vi "LoadMouseLUT.vi"(11 "Metadata":T3[](array[typedef])) -> (0 "error out":errorcluster)   [LabVIEW 2026, in "dependencies.lvlib"]
uses:
  dependencies.lvlib
  MouseLUTSelector.ctl
  KeyboardAndMouseDataAcquisition.ctl
  KeyType.ctl
panel:
  out "Axis Info Debug":T1(array[cluster])
  out "Button Info Debug":T2(array[cluster])
  # "wqeeeeeeeeeeeeeeeeeeeeeeeeeeeeeeeeeeeeeeeeeeeeeeeeeeeeeeeeeeeeeeeeeeeeeeeeeeeeee"
  # "sssssssssssssddddddddddddddddddddddddddddddddddddddddddd"
  # "fsdsdsdsdsdsdsdsdsdsdaaaaaaaaaaaaaaaaaaaaaaaaaaaaaaaaa"
  # "qweeeeeeeeewqqqqqqqqqqqqqqqqqqqqqqqqqqqqqqqqqqqqqqqqqq"
  # "sdffffffffffffffffffAAAAAA"
  # "sdsdsdsdsdsdsdsdsdsdaaaaaaaaaaaaaaaaaaaaaaaaaaaaaaaaaaaaaaaaaaaaaaaaaaaaaaaaaaa"
  # "rewwwwwwwwwwwwwwwwwwwwrewwerrrrrrrrrewwwwwwwwwwwwww"
  # "rew"
  # "rrrrrrrrreeeeeeeewwwwwwwwww"
  # "rrrrrrrreeeeeeeeeeewwwwwwwwwwwwwww"
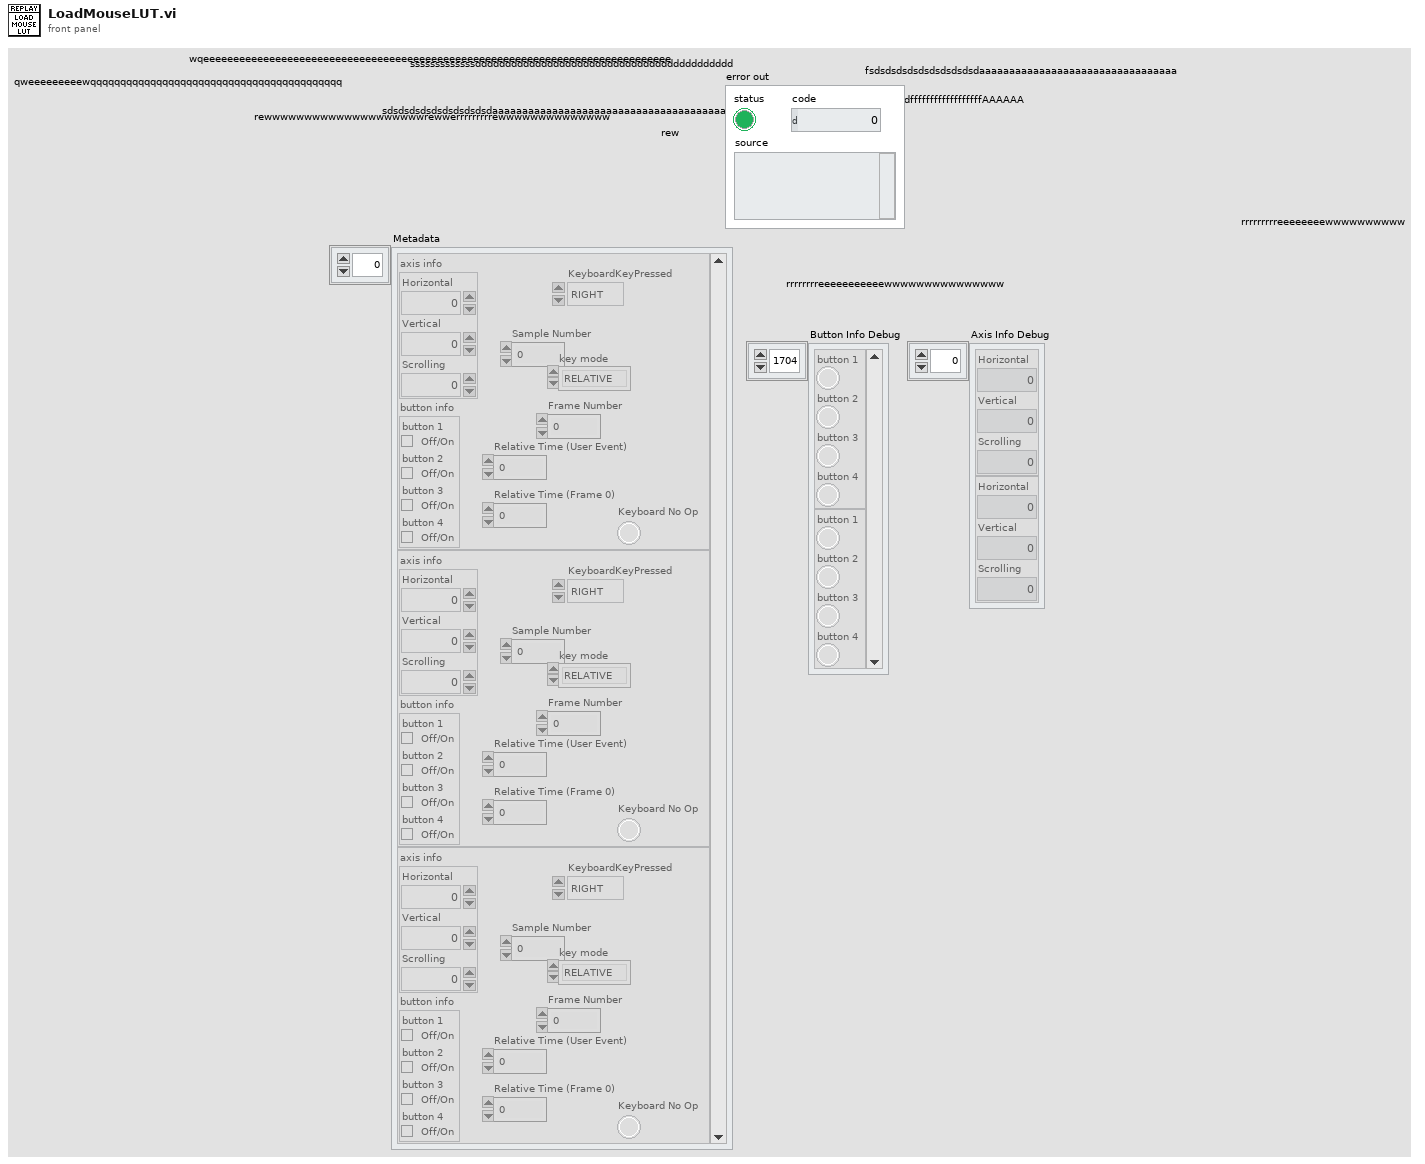
[diagram p1: front panel]
types:
  T1 = cluster{"Horizontal":i32, "Vertical":i32, "Scrolling":i32}[]
  T2 = cluster{"button 1":bool, "button 2":bool, "button 3":bool, "button 4":bool}[]
  T3 = typedef "dependencies.lvlib/KeyboardAndMouseDataAcquisition.ctl" = cluster{"axis info":cluster{"Horizontal":i32, "Vertical":i32, "Scrolling":i32}, "button info":cluster{"button 1":bool, "button 2":bool, "button 3":bool, "button 4":bool}, "Relative Time (User Event)":dbl, "Sample Number":u32, "Relative Time (Frame 0)":dbl, "key mode":enum16{"RELATIVE", "ABSOLUTE"}, "Frame Number":u32, "KeyboardKeyPressed":T4, "Keyboard No Op":bool}
  T4 = typedef "dependencies.lvlib/KeyType.ctl" = enum16{"0", "1", "2", "3", "4", "5", "6", "7", "8", "9", "A", "B", "C", "D", "E", "F", "G", "H", "I", "J", "K", "L", "M", "N", "O", "P", "Q", "R", "S", "T", "U", "V", "W", "X", "Y", "Z", "F1", "F2", "F3", "F4", "F5", "F6", "F7", "F8", "F9", "F10", "F11", "F12", "F13", "F14", "F15", "ADD", "BACK", "BACKSLASH", "CAPITAL", "COMMA", "DECIMAL", "DELETE", "DIVIDE", "DOWN", "END", "EQUALS", "ESCAPE", "GRAVE (`)", "HOME", "INSERT", "LBRACKET", "LCONTROL", "LEFT", "L ALT", "LSHIFT", "LWIN", "MINUS", "MULTIPLY", "NEXT", "NUMLOCK", "NUMPAD_0", "NUMPAD_1", "NUMPAD_2", "NUMPAD_3", "NUMPAD_4", "NUMPAD_5", "NUMPAD_6", "NUMPAD_7", "NUMPAD_8", "NUMPAD_9", "PAUSE", "PERIOD", "PRIOR (PG UP)", "RBRACKET", "RCONTROL", "RETURN", "RIGHT", "R ALT", "RSHIFT", "RWIN", "SCROLL", "SEMICOLON", "SLASH", "SPACE", "SUBTRACT", "TAB", "UP", "ENTER (num pad)", "' (quote)"}
  T5 = typedef "dependencies.lvlib/MouseLUTSelector.ctl" = enum16{"Initialize", "Get Button and Axis Info", "Assign Button and Axis Info to Sample Number"}
  T6 = cluster{"Horizontal":i32, "Vertical":i32, "Scrolling":i32}
  T7 = cluster{"button 1":bool, "button 2":bool, "button 3":bool, "button 4":bool}
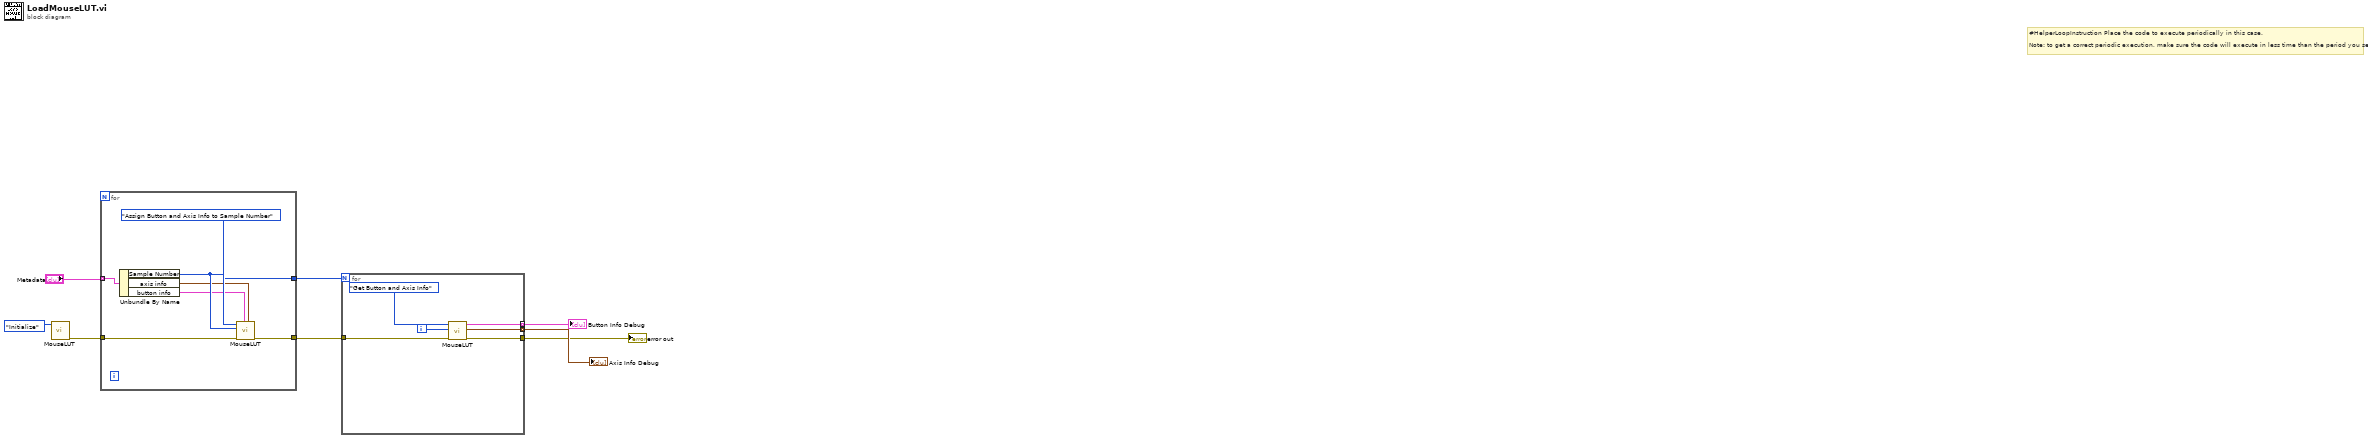
[diagram p0: block diagram]
diagram:
  # "#HelperLoopInstruction Place the code to execute periodically in this case.\n\nNote: to get a correct periodic execution, make sure the code will execute in less time than the period you set."
  n1 = call "MouseLUT.vi"("LUT Selector"=MouseLUTSelector."Initialize") -> ("error out"=w6:errorcluster)  [unwired: 8 in, 2 out]
  n2 = for {
    tunnel: "Metadata" -> [w15] mode=indexing
    tunnel: w6 -> [w14]
    tunnel: [w13] -> w5
    tunnel: [w11] -> w7
    n3 = Unbundle By Name(w15) -> ("Sample Number"=w11:u32, "axis info"=w9:T6, "button info"=w10:T7)
    n4 = call "MouseLUT.vi"("axis info"=w9, "button info"=w10, "error in (no error)"=w14, "Sample Number"=w11, "LUT Selector"=MouseLUTSelector."Assign Button and Axis Info to Sample Number") -> ("error out"=w13:errorcluster)  [unwired: 4 in, 2 out]
  }
  n5 = for {
    N: w7 -> [_]
    tunnel: [w18] -> w1
    tunnel: w5 -> [w21]
    tunnel: [w17] -> w3 mode=indexing
    tunnel: [w16] -> w2 mode=indexing
    i -> [w20]
    n6 = call "MouseLUT.vi"("error in (no error)"=w21, "Sample Number"=w20, "LUT Selector"=MouseLUTSelector."Get Button and Axis Info") -> ("error out"=w18:errorcluster, "axis info out"=w16:T6, "button info out"=w17:T7)  [unwired: 6 in]
  }
  "Button Info Debug" <- w3
  "Axis Info Debug" <- w2
  "error out" <- w1
